vi "TakeWindowScreenshot.vi"(0 "JPEG Image File Path":path, 11 "Error In":errorcluster) -> (15 "Error Out":errorcluster)   [LabVIEW 2019, in "Drona.lvlib"]
doc: "This VI takes screenshot of the primary window and store it in the given file location"
uses:
  Drona.lvlib
  System.Windows.Forms
  System.Drawing
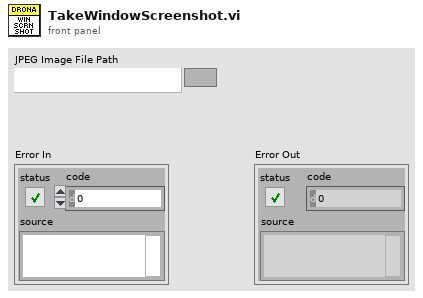
[diagram p1: front panel]
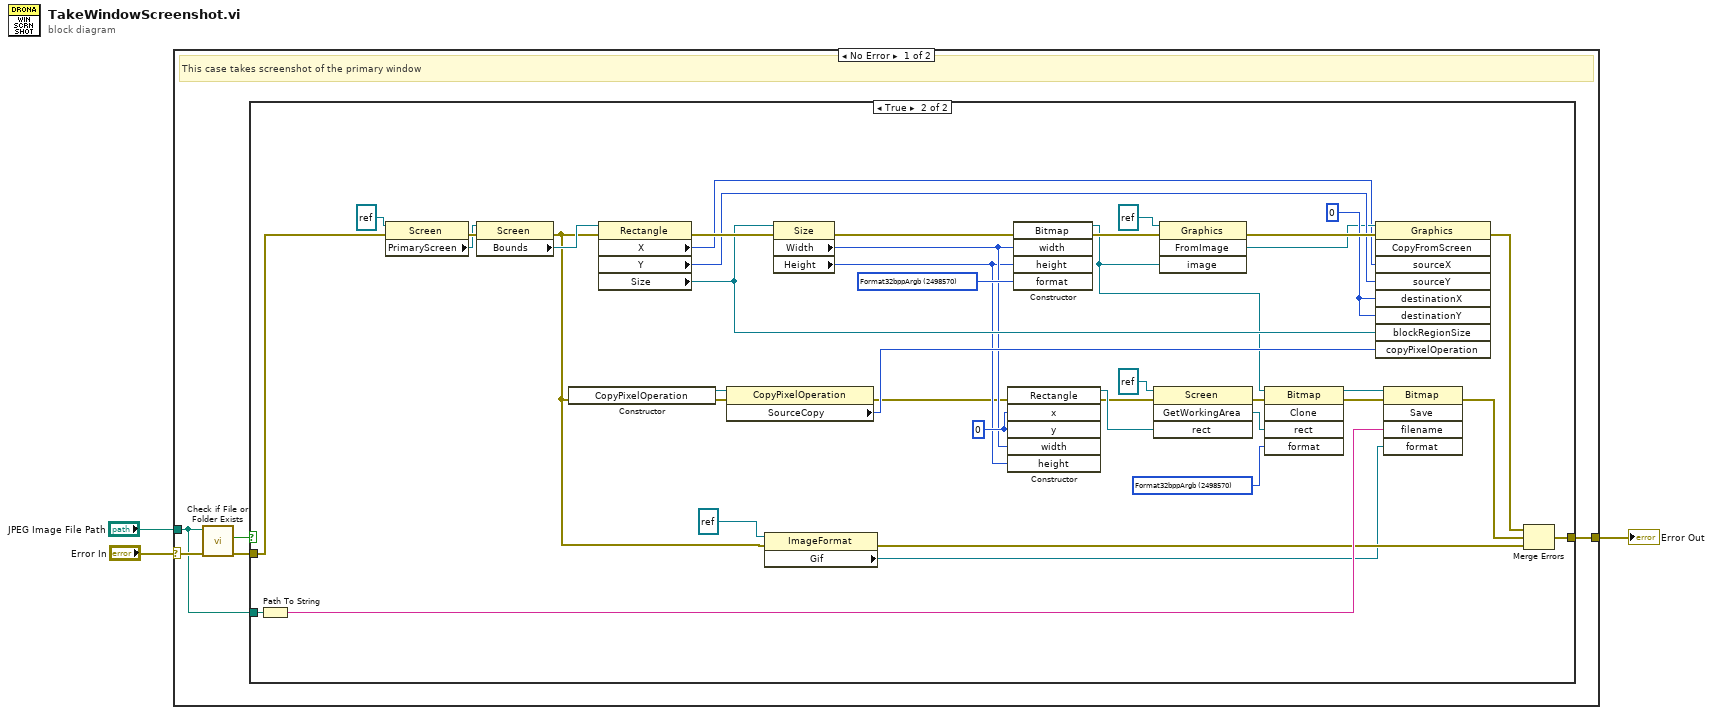
[diagram p0: block diagram]
diagram:
  n1 = case shown="No Error" "Error In" {
    selector: "Error In" -> [w5 w51]
    tunnel: [w8 w51] -> w2
    tunnel: "JPEG Image File Path" -> [w4 _]
    frame No Error {
      # "This case takes screenshot of the primary window"
      n2 = call <vilib>:"Check if File or Folder Exists.vi"("error in (no error)"=w5, "path"=w4) -> ("error out"=w7:errorcluster, "file or folder exists?"=w6:bool)  [unwired: 7 in, 1 out]
      n3 = case shown="True" w6 {
        tunnel: w7 -> [w9 w16]
        tunnel: [w9 w10] -> w8
        tunnel: w4 -> [_ w50]
        frame False {
        }
        frame True {
          w29 = 2498570 items=["DontCare, Undefined"=0, "Max"=15, "Indexed"=65536, "Gdi"=131072, "Format16bppRgb555"=135173, "Format16bppRgb565"=135174, "Format24bppRgb"=137224, "Format32bppRgb"=139273, "Format1bppIndexed"=196865, "Format4bppIndexed"=197634, "Format8bppIndexed"=198659, "Alpha"=262144, "Format16bppArgb1555"=397319, "PAlpha"=524288, "Format32bppPArgb"=925707, "Extended"=1048576, "Format16bppGrayScale"=1052676, "Format48bppRgb"=1060876, "Format64bppPArgb"=1851406, "Canonical"=2097152, "Format32bppArgb"=2498570, "Format64bppArgb"=3424269] ("format")
          w33 = 0 ("x")
          w39 = 0 ("destinationX")
          w48 = 2498570 items=["DontCare, Undefined"=0, "Max"=15, "Indexed"=65536, "Gdi"=131072, "Format16bppRgb555"=135173, "Format16bppRgb565"=135174, "Format24bppRgb"=137224, "Format32bppRgb"=139273, "Format1bppIndexed"=196865, "Format4bppIndexed"=197634, "Format8bppIndexed"=198659, "Alpha"=262144, "Format16bppArgb1555"=397319, "PAlpha"=524288, "Format32bppPArgb"=925707, "Extended"=1048576, "Format16bppGrayScale"=1052676, "Format48bppRgb"=1060876, "Format64bppPArgb"=1851406, "Canonical"=2097152, "Format32bppArgb"=2498570, "Format64bppArgb"=3424269] ("format")
          n4 = Path To String(path=w50) -> (string=w13:string)
          n5 = property class="Screen"(reference=refnum<k24> refnum ("référence"), error in=w16) -> (error out=w45:errorcluster, "PrimaryScreen"=w44:refnum<k24>)  [unwired: 1 out]
          n6 = property class="Screen"(reference=w44, error in=w45) -> (error out=w15:errorcluster, "Bounds"=w43:refnum<k24>)  [unwired: 1 out]
          n7 = constructor class="CopyPixelOperation"(error in=w15) -> (reference out=w38:refnum<k24>, error out=w37:errorcluster)  [unwired: 2 in, 1 out]
          n8 = property class="Rectangle"(reference=w43, error in=w15) -> (error out=w42:errorcluster, "X"=w24:i32, "Y"=w40:i32, "Size"=w34:refnum<k24>)  [unwired: 1 out]
          n9 = property class="CopyPixelOperation"(reference=w38, error in=w37) -> (error out=w19:errorcluster, "SourceCopy"=w36:i32)  [unwired: 1 out]
          n10 = property class="ImageFormat"(reference=refnum<k24> refnum ("référence"), error in=w15) -> (error out=w12:errorcluster, "Gif"=w11:refnum<k24>)  [unwired: 1 out]
          n11 = property class="Size"(reference=w34, error in=w42) -> (error out=w23:errorcluster, "Width"=w28:i32, "Height"=w27:i32)  [unwired: 1 out]
          n12 = constructor class="Rectangle"(error in=w19, "x"=w33, "y"=w33, "width"=w28, "height"=w27) -> (reference out=w31:refnum<k24>, error out=w21:errorcluster)  [unwired: 2 in, 5 out]
          n13 = constructor class="Bitmap"(error in=w23, "width"=w28, "height"=w27, "format"=w48) -> (reference out=w26:refnum<k24>, error out=w47:errorcluster)  [unwired: 2 in, 4 out]
          n14 = invoke class="Screen" method="GetWorkingArea"(reference=refnum<k24> refnum ("référence"), error in=w21, "rect"=w31) -> (error out=w22:errorcluster, "GetWorkingArea"=w30:refnum<k24>)  [unwired: 1 in, 2 out]
          n15 = invoke class="Graphics" method="FromImage"(reference=refnum<k24> refnum ("référence"), error in=w47, "image"=w26) -> (error out=w41:errorcluster, "FromImage"=w35:refnum<k24>)  [unwired: 1 in, 2 out]
          n16 = invoke class="Bitmap" method="Clone"(reference=w26, error in=w22, "rect"=w30, "format"=w29) -> (reference out=w25:refnum<k24>, error out=w20:errorcluster)  [unwired: 1 in, 3 out]
          n17 = invoke class="Graphics" method="CopyFromScreen"(reference=w35, error in=w41, "sourceX"=w24, "sourceY"=w40, "destinationX"=w39, "destinationY"=w39, "blockRegionSize"=w34, "copyPixelOperation"=w36) -> (error out=w18:errorcluster)  [unwired: 1 in, 8 out]
          n18 = invoke class="Bitmap" method="Save"(reference=w25, error in=w20, "filename"=w13, "format"=w11) -> (error out=w17:errorcluster)  [unwired: 1 in, 4 out]
          n19 = Merge Errors(w18, w17, w12) -> (w10:errorcluster)
        }
      }
    }
    frame Error {
      # "If error, this case pass that error message only"
    }
  }
  "Error Out" <- w2
